vi "AI_Evaluate_Point.vi"(0 "Grid":enum8{"Empty", "Black", "White"}[][](array[ring])=[[enum."Empty", enum."Empty", enum."Empty", enum."Empty", enum."Empty", enum."Empty", enum."Empty", enum."Empty", enum."Empty", enum."Empty", enum."Empty", enum."Empty", enum."Empty", enum."Empty", enum."Empty"], [enum."Empty", enum."Empty", enum."Empty", enum."Empty", enum."Empty", enum."Empty", enum."Empty", enum."Empty", enum."Empty", enum."Empty", enum."Empty", enum."Empty", enum."Empty", enum."Empty", enum."Empty"], [enum."Empty", enum."Empty", enum."Empty", enum."Empty", enum."Empty", enum."Empty", enum."Empty", enum."Empty", enum."Empty", enum."Empty", enum."Empty", enum."Empty", enum."Empty", enum."Empty", enum."Empty"], [enum."Empty", enum."Empty", enum."Empty", enum."Empty", enum."Empty", enum."Empty", enum."Empty", enum."Empty", enum."Empty", enum."Empty", enum."Empty", enum."Empty", enum."Empty", enum."Empty", enum."Empty"], [enum."Empty", enum."Empty", enum."Empty", enum."Empty", enum."Empty", enum."Empty", enum."Empty", enum."Empty", enum."Empty", enum."Empty", enum."Empty", enum."Empty", enum."Empty", enum."Empty", enum."Empty"], [enum."Empty", enum."Empty", enum."Empty", enum."Empty", enum."Empty", enum."Empty", enum."Empty", enum."Empty", enum."Empty", enum."Empty", enum."Empty", enum."Empty", enum."Empty", enum."Empty", enum."Empty"], [enum."Empty", enum."Empty", enum."Empty", enum."Empty", enum."Empty", enum."Empty", enum."Empty", enum."Empty", enum."Empty", enum."Empty", enum."Empty", enum."Empty", enum."Empty", enum."Empty", enum."Empty"], [enum."Empty", enum."Empty", enum."Empty", enum."Empty", enum."Empty", enum."Empty", enum."Empty", enum."Empty", enum."Empty", enum."Empty", enum."Empty", enum."Empty", enum."Empty", enum."Empty", enum."Empty"], [enum."Empty", enum."Empty", enum."Empty", enum."Empty", enum."Empty", enum."Empty", enum."Empty", enum."Empty", enum."Empty", enum."Empty", enum."Empty", enum."Empty", enum."Empty", enum."Empty", enum."Empty"], [enum."Empty", enum."Empty", enum."Empty", enum."Empty", enum."Empty", enum."Empty", enum."Empty", enum."Empty", enum."Empty", enum."Empty", enum."Empty", enum."Empty", enum."Empty", enum."Empty", enum."Empty"], [enum."Empty", enum."Empty", enum."Empty", enum."Empty", enum."Empty", enum."Empty", enum."Empty", enum."Empty", enum."Empty", enum."Empty", enum."Empty", enum."Empty", enum."Empty", enum."Empty", enum."Empty"], [enum."Empty", enum."Empty", enum."Empty", enum."Empty", enum."Empty", enum."Empty", enum."Empty", enum."Empty", enum."Empty", enum."Empty", enum."Empty", enum."Empty", enum."Empty", enum."Empty", enum."Empty"], [enum."Empty", enum."Empty", enum."Empty", enum."Empty", enum."Empty", enum."Empty", enum."Empty", enum."Empty", enum."Empty", enum."Empty", enum."Empty", enum."Empty", enum."Empty", enum."Empty", enum."Empty"], [enum."Empty", enum."Empty", enum."Empty", enum."Empty", enum."Empty", enum."Empty", enum."Empty", enum."Empty", enum."Empty", enum."Empty", enum."Empty", enum."Empty", enum."Empty", enum."Empty", enum."Empty"], [enum."Empty", enum."Empty", enum."Empty", enum."Empty", enum."Empty", enum."Empty", enum."Empty", enum."Empty", enum."Empty", enum."Empty", enum."Empty", enum."Empty", enum."Empty", enum."Empty", enum."Empty"]], 5 "Move":T1={"Row"=7, "Col"=7, "Stone"=enum."Black"}, 11 "error in":errorcluster) -> (4 "Score":dbl, 15 "error out":errorcluster)   [LabVIEW 2026]
doc: "한 칸 평가: Move.Stone을 (Row,Col)에 둔다고 가정하고 4방향 연속 길이와 열린 끝 수로 점수를 합산.\n5목=100000, 열린4=10000, 닫힌4=1000, 열린3=1000, 닫힌3=100, 열린2=100, 닫힌2=10, 막힌 쪽 0."
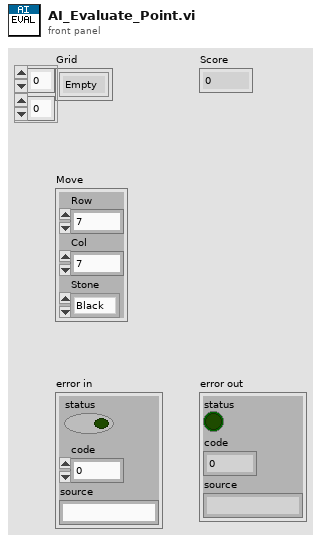
[diagram p1: front panel]
types:
  T1 = cluster{"Row":i32, "Col":i32, "Stone":enum8{"Empty", "Black", "White"}}
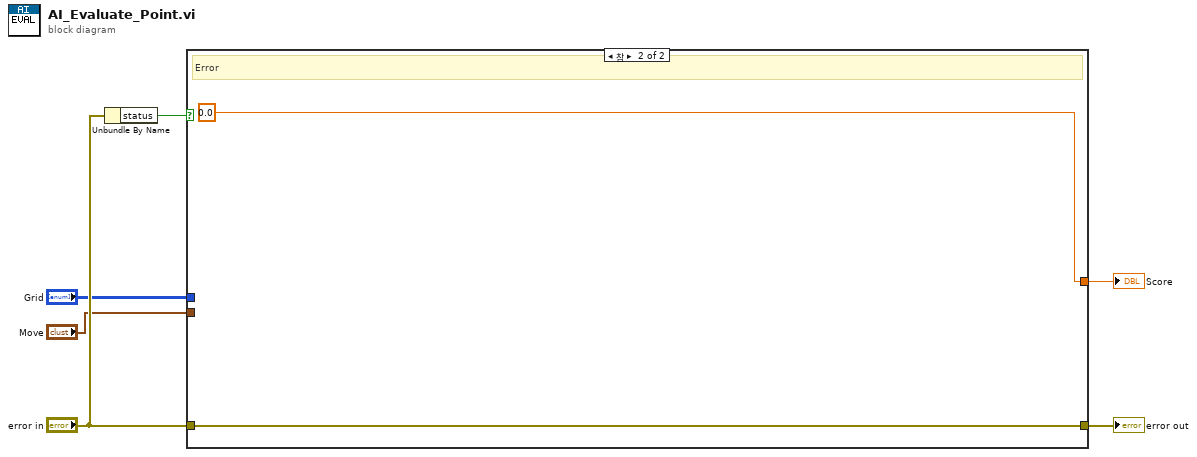
[diagram p0: block diagram]
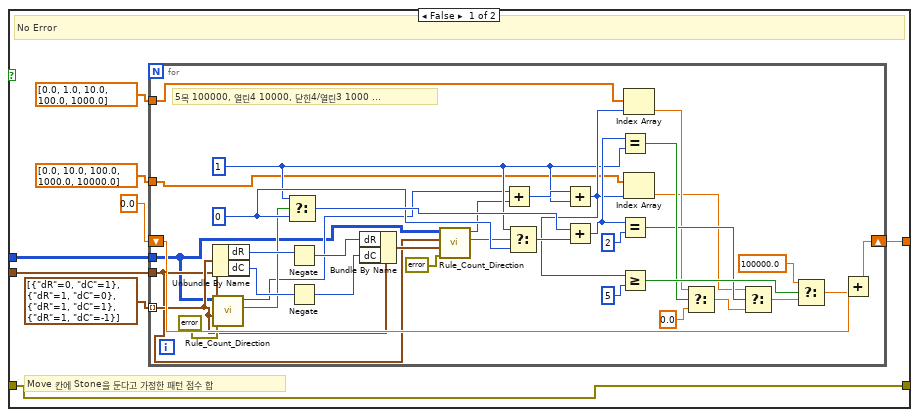
[diagram p2: hidden frame]
diagram:
  n1 = Unbundle By Name("error in") -> ("status"=w4:bool)
  n2 = case shown="참" w4 {
    tunnel: "Grid" -> [w7 _]
    tunnel: "Move" -> [w8 _]
    tunnel: "error in" -> [w9 w52]
    tunnel: [w14 0.0] -> w5
    tunnel: [w9 w52] -> w6
    frame False {
      # "Move 칸에 Stone을 둔다고 가정한 패턴 점수 합"
      # "No Error"
      n3 = for {
        tunnel: dbl[] [0.0, 10.0, 100.0, 1000.0, 10000.0] ("Open Both") -> [w17]
        tunnel: dbl[] [0.0, 1.0, 10.0, 100.0, 1000.0] ("Open One") -> [w18]
        tunnel: cluster{"dR":i32, "dC":i32}[] [{"dR"=0, "dC"=1}, {"dR"=1, "dC"=0}, {"dR"=1, "dC"=1}, {"dR"=1, "dC"=-1}] ("Directions") -> [w19] mode=indexing
        shift-right: [w50] -> w14
        shift-left: 0.0 -> [w51]
        tunnel: w7 -> [w15]
        tunnel: w8 -> [w16]
        w32 = 0
        w31 = 1
        # "5목 100000, 열린4 10000, 닫힌4/열린3 1000 ..."
        n4 = Unbundle By Name(w19) -> ("dR"=w23:i32, "dC"=w24:i32)
        n5 = call "Rule_Count_Direction.vi"("error in"=errorcluster {"status"=FALSE, "code"=0, "source"=""}, "Direction"=w19, "Move"=w16, "Grid"=w15) -> ("Open End"=w22:bool, "Count"=w21:i32)  [unwired: 5 in, 1 out]
        n6 = Select(t=w31, s=w22, f=w32) -> (s? t:f=w35:i32)
        n7 = Negate(x=w23) -> (-x=w25:i32)
        n8 = Negate(x=w24) -> (-x=w26:i32)
        n9 = Bundle By Name(cluster=w19, "dR"=w25, "dC"=w26) -> (w27:cluster{"dR":i32, "dC":i32})
        n10 = call "Rule_Count_Direction.vi"("error in"=errorcluster {"status"=FALSE, "code"=0, "source"=""}, "Direction"=w27, "Move"=w16, "Grid"=w15) -> ("Open End"=w30:bool, "Count"=w29:i32)  [unwired: 5 in, 1 out]
        n11 = Add(x=w21, y=w29) -> (x+y=w33:i32)
        n12 = Select(t=w31, s=w30, f=w32) -> (s? t:f=w36:i32)
        n13 = Add(x=w33, y=w31) -> (x+y=w34:i32)
        n14 = Add(x=w35, y=w36) -> (x+y=w37:i32)
        n15 = Equal?(x=w37, y=w31) -> (x = y?=w43:bool)
        n16 = Equal?(x=w37, y=2) -> (x = y?=w42:bool)
        n17 = Greater Or Equal?(x=w34, y=5) -> (x >= y?=w47:bool)
        n18 = Index Array(array=w18, index=w34) -> (element=w39:dbl)
        n19 = Index Array(array=w17, index=w34) -> (element=w38:dbl)
        n20 = Select(t=w39, s=w43, f=0.0) -> (s? t:f=w44:dbl)
        n21 = Select(t=w38, s=w42, f=w44) -> (s? t:f=w45:dbl)
        n22 = Select(t=100000.0, s=w47, f=w45) -> (s? t:f=w49:dbl)
        n23 = Add(x=w51, y=w49) -> (x+y=w50:dbl)
      }
    }
    frame True {
      # "Error"
    }
  }
  "Score" <- w5
  "error out" <- w6
